vi "Analog_Write_Ex.vi"() -> ()   [LabVIEW 2026]
panel:
  in  "Valor":u8(slide) scale=0.0..255.0
  in  "Canal":u8
  in  "VISA resource name":refnum<visa-resource-name>
  in  "Stop Button":bool
  out "error out":errorcluster
  # "Ejemplo: Analog Write"
  # "Descripción: Escribe un valor analógico en un pin de salida del microcontrolador."
  # "Configuracion"
  # "Indicadores"
  # "Control"
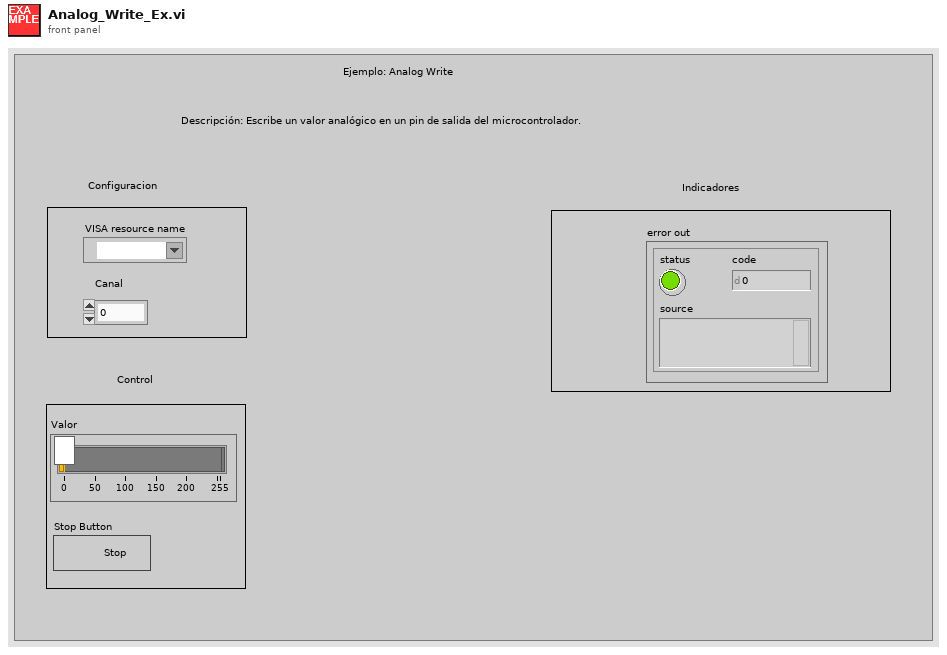
[diagram p1: front panel]
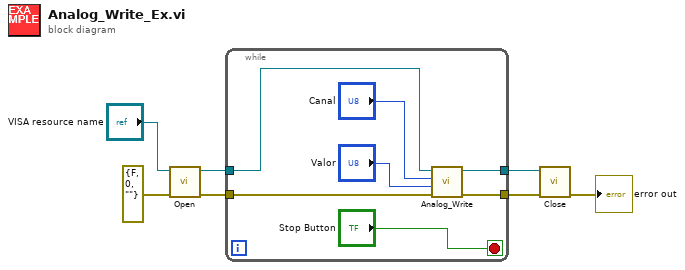
[diagram p0: block diagram]
diagram:
  n1 = call "Open.vi"("error in (no error)"=errorcluster {"status"=FALSE, "code"=0, "source"=""}, "VISA resource name"="VISA resource name") -> ("error out"=w7:errorcluster, "VISA resource name out"=w6:refnum<visa-resource-name>)  [unwired: 8 in]
  n2 = while {
    tunnel: w6 -> [w11]
    tunnel: w7 -> [w10]
    tunnel: [w13] -> w2
    tunnel: [w12] -> w1
    stop <- "Stop Button" stop-if-true
    n3 = call "Analog_Write.vi"("error in (no error)"=w10, "Valor"="Valor", "Canal"="Canal", "VISA resource name"=w11) -> ("error out"=w12:errorcluster, "VISA resource name out"=w13:refnum<visa-resource-name>)  [unwired: 6 in]
  }
  n4 = call "Close.vi"("error in (no error)"=w1, "VISA resource name"=w2) -> ("error out"=→"error out":errorcluster)  [unwired: 9 in]
